vi "Main Editor UI.vi"() -> ()   [LabVIEW 2014, in "Shared Memory editor node.lvclass"]
doc: "This is the main view for configuration the behavior of a module in the DCAF standard editor."
uses:
  Shared Memory editor node.lvclass
  <vilib>/NI/Configuration Framework/Node/NodeRef.ctl
  <vilib>/NI/Configuration Framework/Node/NISE_CEF_Node.lvclass
  <vilib>/NI/AMC/Message Queue.ctl
  <vilib>/NI/AMC/Message.ctl
  <vilib>/NI/Tools/Keyed Array/KeyedArray.ctl
  <vilib>/NI/Configuration Framework/Node/UserEventRef.ctl
  <vilib>/NI/Configuration Framework/Controls/EventCluster.ctl
  <vilib>/NI/DCAF UI Toolkit/Controls/Configure.ctl
  <vilib>/NI/DCAF UI Toolkit/Controls/Add.ctl
  <vilib>/NI/DCAF UI Toolkit/Controls/Remove.ctl
  <vilib>/NI/Configuration Framework/Node/StopEvent.ctl
  <vilib>/NI/Configuration Framework/Node/RefreshUIEvent.ctl
  <vilib>/NI/Configuration Framework/Node/CacheState.ctl
  <vilib>/NI/Configuration Framework/Node/NodeChangeEvent.ctl
  <vilib>/NI/Tag Bus/tag/Data Type.ctl
  Permissions Enum.ctl
  <vilib>/NI/DCAF/Tag Editor Core/Table API/Available Tag Menu/channel action event.ctl
  <vilib>/NI/DCAF/Tag Editor Core/Table API/Available Tag Menu/dialog output action.ctl
  <vilib>/NI/Tag Bus Module Framework/channel/TBM channel.lvclass
  <vilib>/NI/Tag Bus/tag/tag descriptor.lvclass
  <vilib>/NI/DCAF/Tag Editor Core/Table API/Table Manager/Call Back Ref Type Def.ctl
  <vilib>/NI/DCAF/Tag Editor Core/Configuration Editor/Classes/Engine Parent/Engine Parent Editor Node.lvclass
  <vilib>/NI/DCAF/Tag Editor Core/Configuration Editor/Classes/Module editor node/module editor node.lvclass
  sync/sync item.ctl
  sync/sync mechanism.ctl
  <vilib>/NI/DCAF UI Toolkit/Controls/Move One Left.ctl
  <vilib>/NI/DCAF UI Toolkit/Controls/Move One Right.ctl
  <vilib>/NI/DCAF/Tag Editor Core/Table API/Table Manager/references.ctl
  ui controls sync.ctl
  ui controls config.ctl
  ui controls header.ctl
  <vilib>/NI/Tag Bus Module Framework/channel/channel classification.ctl
  <vilib>/Utility/miscctls.llb/LVPositionTypeDef.ctl
  <vilib>/NI/DCAF/Tag Editor Core/Configuration Editor/Classes/Engine Parent/read engine configuration.vi
  <vilib>/NI/Module Execution Interface/Engine Configuration/engine configuration.lvclass
  <vilib>/NI/DCAF/Tag Editor Core/Table API/Listbox/Multi Column Listbox.lvclass
  <vilib>/NI/Configuration Framework/NISE_CEF_TreeControl.lvlib
  <vilib>/NI/Tools/Keyed Array/Tools_KeyedArray.lvlib
  <vilib>/NI/AMC/AMC.lvlib
  <vilib>/NI/DCAF/Tag Editor Core/Table API/Table Manager.lvlib
  <vilib>/NI/DCAF/Tag Editor Core/Table API/Table Manager/Table Manager.lvclass
  <vilib>/NI/DCAF UI Toolkit/Controls/DCAF UI Elements.lvlib
  module/configuration/Shared Memory configuration.lvclass
panel:
  in  "user event out":refnum<user-event>
  in  "Permissions":T1=enum."Read from Memory"
  in  "data type":T2
  in  "node change":T3
  in  "cache state":T4
  in  "refresh UI":T5
  in  "stop event":T6
  in  "Tab Control":T7(tab)
  in  "to shm list":i32(listbox)
  in  "from shm list":i32(listbox)
  in  "add to":T8
  in  "remove to":T9
  in  "add from":T8
  in  "remove from":T9
  in  "avail tags":i32(listbox)
  in  "View":enum32{"From Shared Memory", "To Shared Memory"}(radio)
  in  "Timeout (us)":u32 step=25
  in  "sync end of cycle":T10[](array[typedef])
  in  "Include start time":bool
  out "Shared memory name":string
  out "Struct prototype":string
  in  "sync start of cycle":T10[](array[typedef])
  out "Struct name":string
  in  "Enable sync":bool
  out "C Header File Preview":string
  out "build":u16
  out "fix":u16
  out "minor":u16
  out "major":u16=1
  in  "Generate Header":bool
  in  "output file path":path caption="Output File Path"
  in  "output file string":string caption="output file string (optional)"
  in  "input file string":string caption="input file string (optional)"
  in  "Remove Button":T12
  in  "Add Button":T13
  in  "Table":i32(listbox)
  in  "settings":T14
  in  "user event":T15
  in  "main queue":T16
  in  "node ref":T17
  # "Start of cycle"
  # "End of cycle (optional response)"
  # "Mechanism"
  # "Name in struct"
  # "Mechanism"
  # "Name in struct"
  # "C Header File Generation"
  # "Version"
  # "Shared Memory Files (<EngineName>_<\"input/output\">_<DataType>_<FileString>)"
  # "The data file names will follow a fixed format with an optional appended user file name string. File input and output classification is from the perspective of an  external process (or application) which will access the file.\n\nExample: A C application running in parallel to the DCAF based LabVIEW Real-Time EXE application will view any file that it writes to as an \"output\" data file in Linux shared memory."
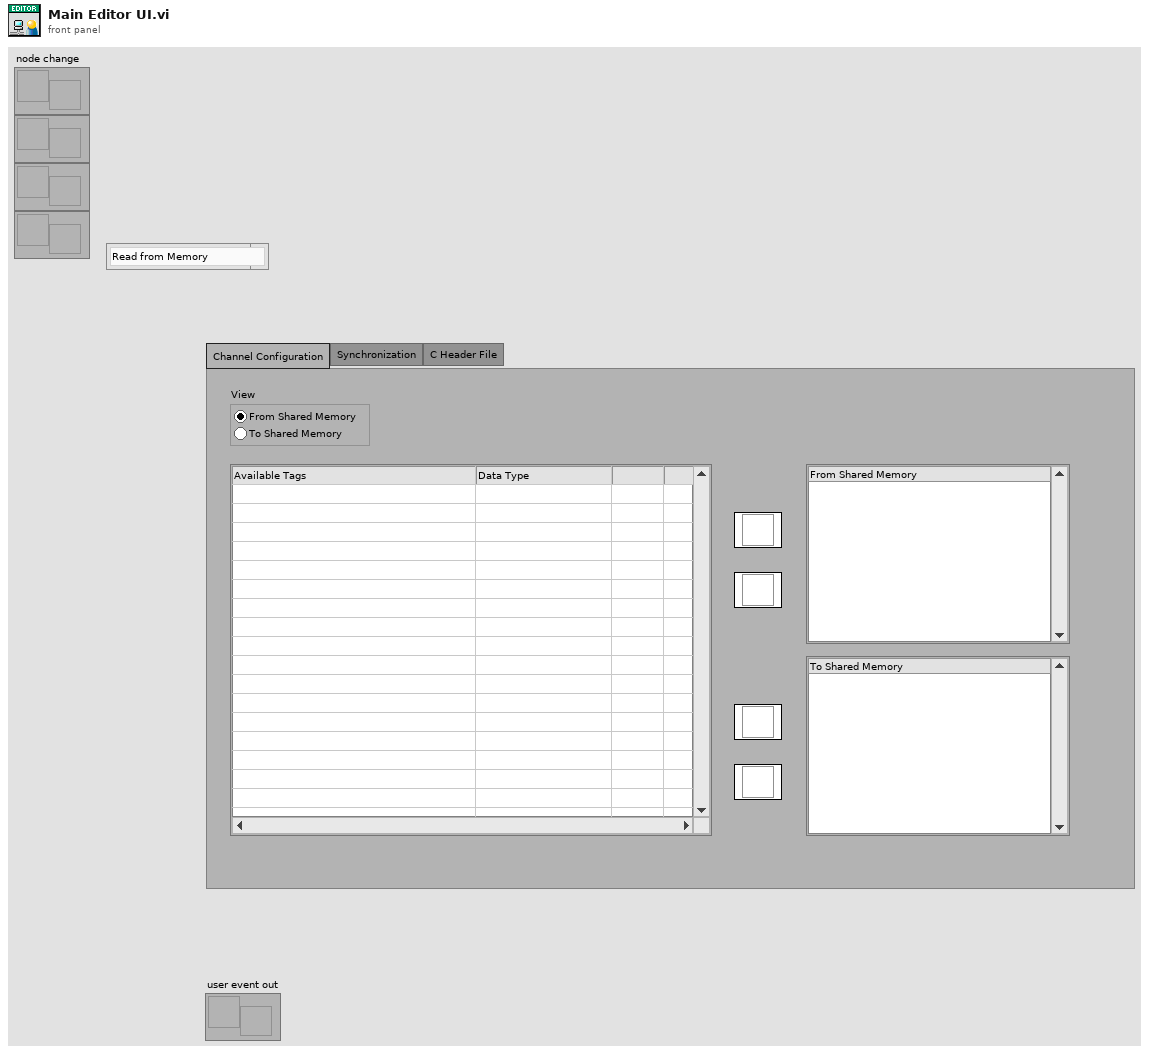
[diagram p1: front panel]
types:
  T1 = typedef "Shared Memory editor node.lvclass/Permissions Enum.ctl" = enum16{"Write to Memory", "Read from Memory"}
  T2 = typedef "tag bus.lvlib/tag descriptor.lvclass/Data Type.ctl" = enum16{"Double", "Single", "I64", "I32", "I16", "I8", "U64", "U32", "U16", "U8", "Boolean", "String", "Array of Double", "Array of Single", "Array of I64", "Array of I32", "Array of I16", "Array of I8", "Array of U64", "Array of U32", "Array of U16", "Array of U8", "Array of Boolean", "Array of String"}
  T3 = typedef "NISE_CEF_Node.lvclass/NodeChangeEvent.ctl" = refnum<user-event>
  T4 = typedef "NISE_CEF_Node.lvclass/CacheState.ctl" = refnum<user-event>
  T5 = typedef "NISE_CEF_Node.lvclass/RefreshUIEvent.ctl" = refnum<user-event>
  T6 = typedef "NISE_CEF_Node.lvclass/StopEvent.ctl" = refnum<user-event>
  T7 = enum32{"Channel Configuration", "Synchronization", "C Header File", "Memory Configuration", "Channel Configuration (old)"}
  T8 = typedef "DCAF UI Elements.lvlib/Move One Right.ctl" = bool
  T9 = typedef "DCAF UI Elements.lvlib/Move One Left.ctl" = bool
  T10 = typedef "Shared Memory configuration.lvclass/sync item.ctl" = cluster{"mechanism":T11, "name":string}
  T11 = typedef "Shared Memory configuration.lvclass/sync mechanism.ctl" = enum16{"Semaphore"}
  T12 = typedef "DCAF UI Elements.lvlib/Remove.ctl" = bool
  T13 = typedef "DCAF UI Elements.lvlib/Add.ctl" = bool
  T14 = typedef "DCAF UI Elements.lvlib/Configure.ctl" = bool
  T15 = typedef "NISE_CEF_Node.lvclass/UserEventRef.ctl" = refnum<user-event>
  T16 = typedef "AMC.lvlib/Message Queue.ctl" = refnum<queue>
  T17 = typedef "NISE_CEF_Node.lvclass/NodeRef.ctl" = refnum<data-value>
  T18 = typedef "Shared Memory editor node.lvclass/ui controls header.ctl" = cluster{"major":refnum<vi>, "minor":refnum<vi>, "fix":refnum<vi>, "build":refnum<vi>, "file path":refnum<vi>, "file preview":refnum<vi>}
  T19 = typedef "Shared Memory editor node.lvclass/ui controls config.ctl" = cluster{"avail tags":refnum<vi>, "from shm list":refnum<vi>, "to shm list":refnum<vi>, "view":refnum<vi>, "add to":refnum<vi>, "add from":refnum<vi>, "remove to":refnum<vi>, "remove from":refnum<vi>}
  T20 = typedef "Shared Memory editor node.lvclass/ui controls sync.ctl" = cluster{"struct name":refnum<vi>, "timeout":refnum<vi>, "shm name":refnum<vi>, "sync end of cycle":refnum<vi>, "sync start of cycle":refnum<vi>, "enable sync":refnum<vi>, "include start time":refnum<vi>, "struct prototype":refnum<vi>}
  T21 = typedef "Table Manager.lvlib/Table Manager.lvclass/references.ctl" = cluster{"stop event":T6, "refresh UI":T5, "cache state":T4, "node change":T3, "user event out":refnum<user-event>, "main queue":T16, "user event":T15}
  T22 = typedef "LVPositionTypeDef.ctl" = cluster{"Left":i32, "Top":i32}
  T23 = typedef "Table Manager.lvlib/Table Manager.lvclass/object ref.ctl" = cluster{"engine":refnum<data-value>, "Node Ref":refnum<data-value>}
  T24 = typedef "Table Manager.lvlib/Column.lvclass/Column Descriptor.ctl" = cluster{"name":string, "caption":string, "Column Type":T25, "Params":string, "AutoSizeMode":i32, "FillWeight":sgl, "MinWidth":u32, "tooltip":string, "Enum Reference":refnum<vi>, "Channel suffix":string, "Read Only":bool, "Call Back VI":T26, "DT Dependency":i32, "name dependency":i32, "data type":T2, "Custom Column":refnum<class "Column.lvclass">}
  T25 = typedef "Table Manager.lvlib/Column.lvclass/Column Type.ctl" = enum16{"String", "Mapping", "Enum", "Custom"}
  T26 = typedef "Table Manager.lvlib/Table Manager.lvclass/Call Back Ref Type Def.ctl" = refnum<vi>
  T27 = typedef "Table Manager.lvlib/Table Manager.lvclass/Table Events.ctl" = cluster{"Menu Selection":refnum<user-event>}
  T28 = typedef "TBM channel.lvclass/channel classification.ctl" = enum16{"input data", "output data", "processing parameter", "processing result"}
  T29 = enum8{"Enabled", "Disabled", "Disabled and Grayed Out"}
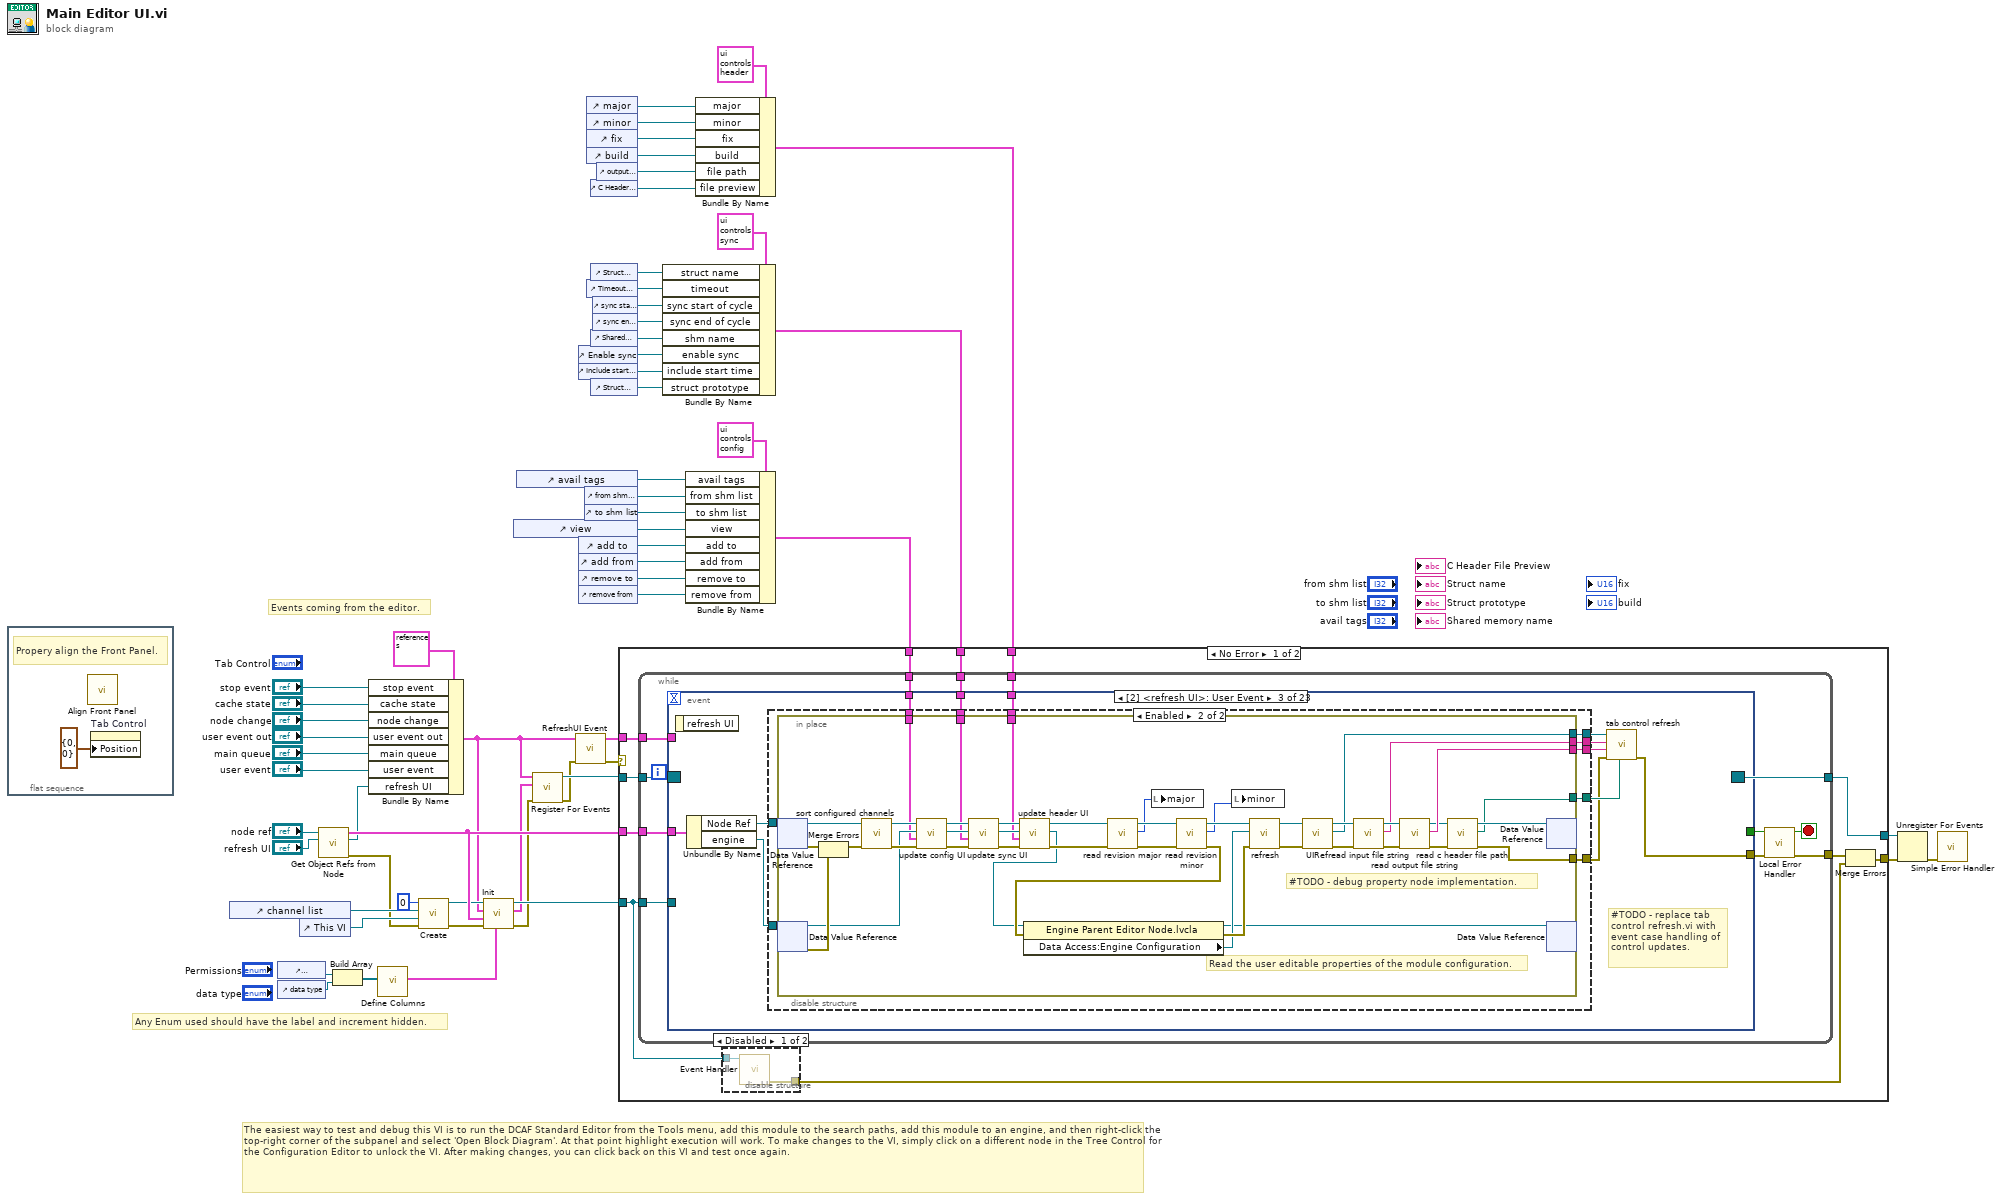
[diagram p0: block diagram]
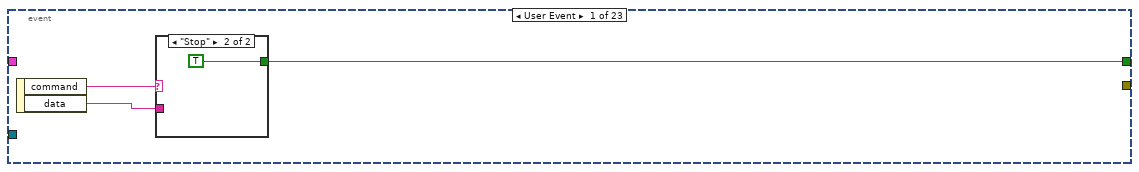
[diagram p3: hidden frame]
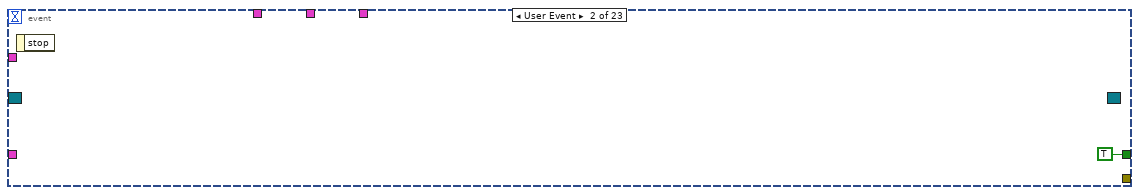
[diagram p5: hidden frame]
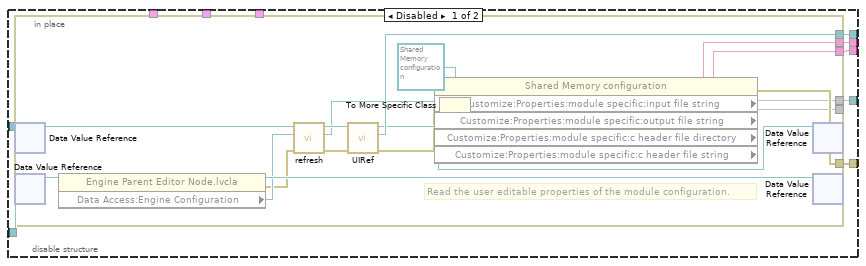
[diagram p6: hidden frame]
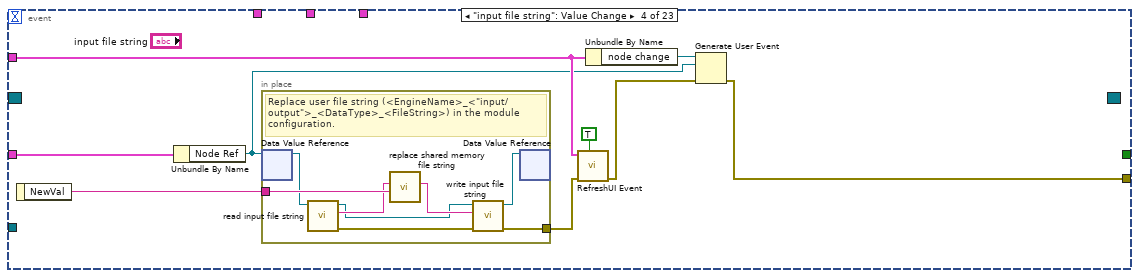
[diagram p7: hidden frame]
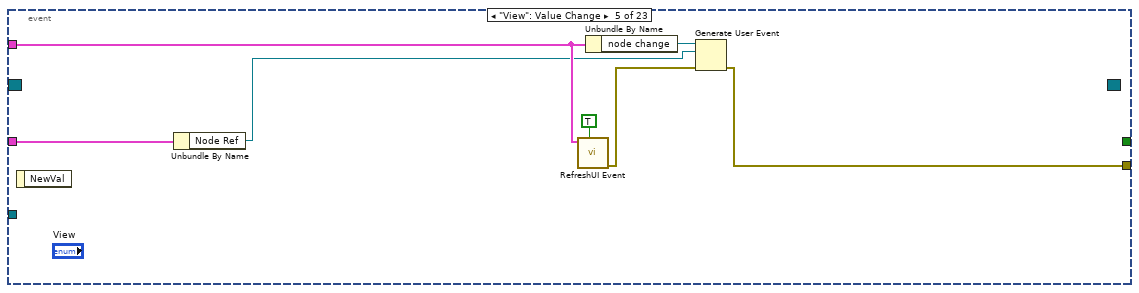
[diagram p8: hidden frame]
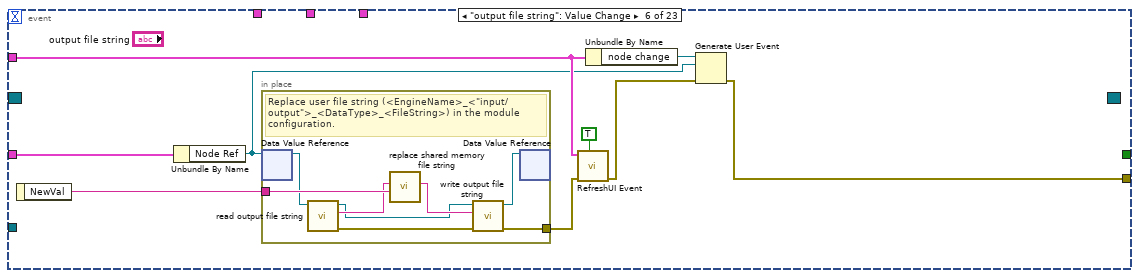
[diagram p9: hidden frame]
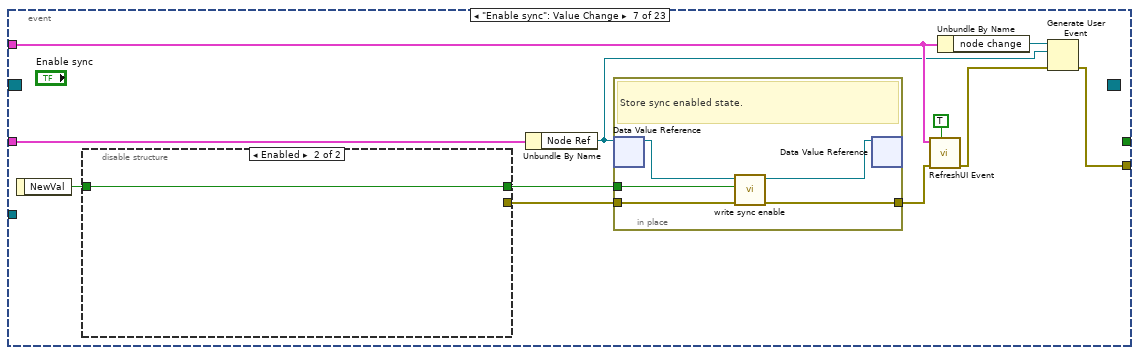
[diagram p10: hidden frame]
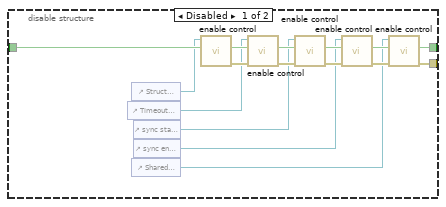
[diagram p11: hidden frame]
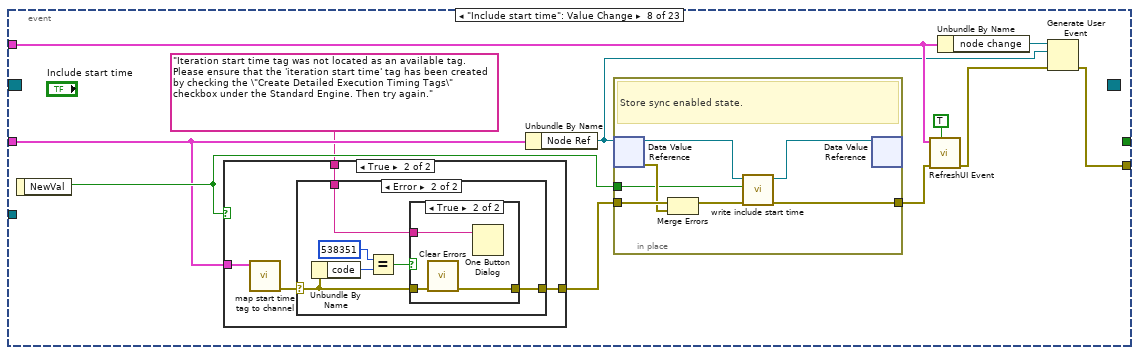
[diagram p12: hidden frame]
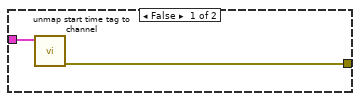
[diagram p13: hidden frame]
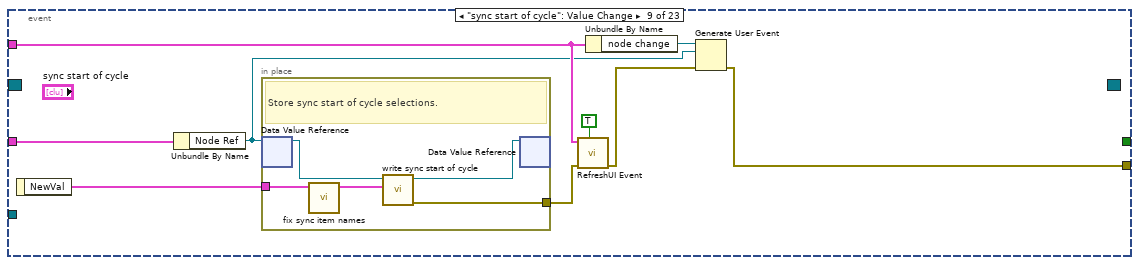
[diagram p16: hidden frame]
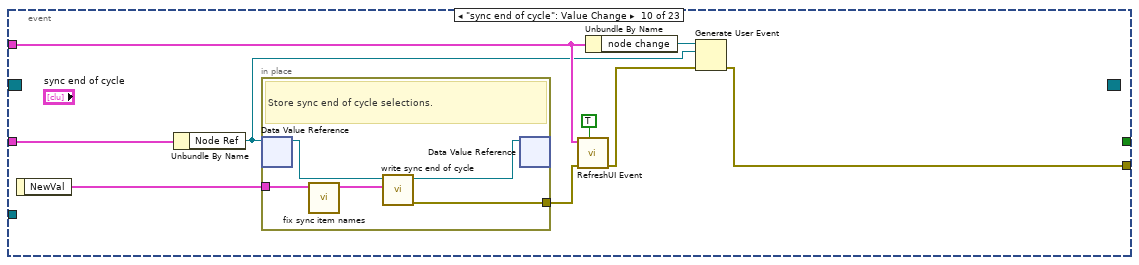
[diagram p17: hidden frame]
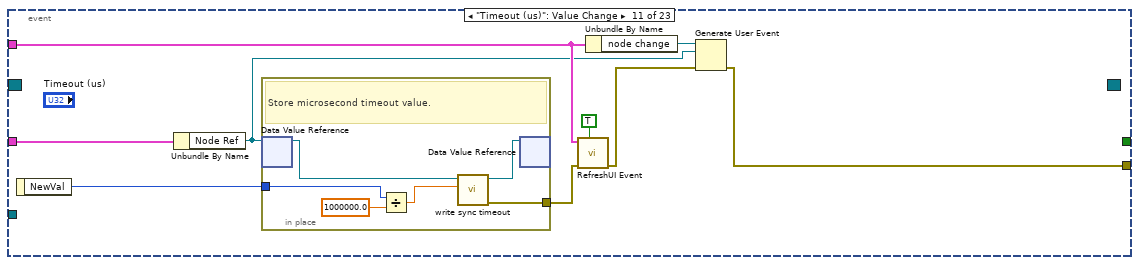
[diagram p18: hidden frame]
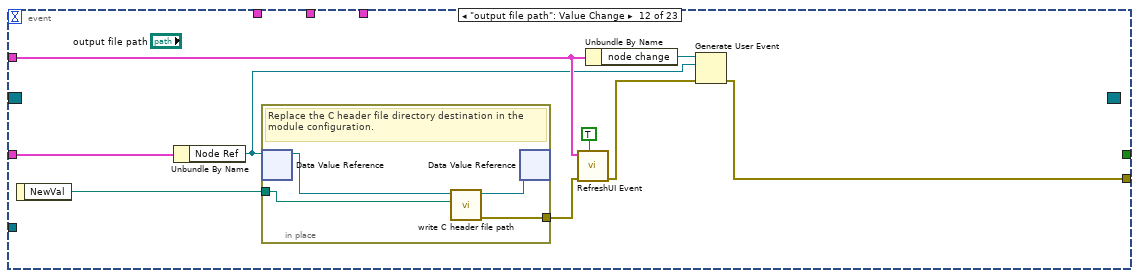
[diagram p19: hidden frame]
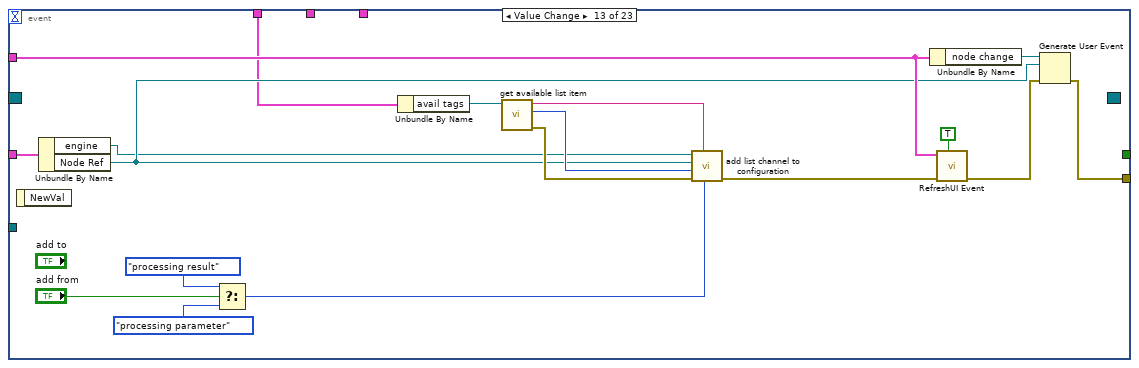
[diagram p20: hidden frame]
diagram:
  # "The easiest way to test and debug this VI is to run the DCAF Standard Editor from the Tools menu, add this module to the search paths, add this module to an engine, and then right-click the top-right corner of the subpanel and select 'Open Block Diagram'. At that point highlight execution will work. To make changes to the VI, simply click on a different node in the Tree Control for the Configuration Editor to unlock the VI. After making changes, you can click back on this VI and test once again."
  # "Any Enum used should have the label and increment hidden."
  # "Events coming from the editor."
  n1 = flat-sequence {
    frame #0 {
      # "Propery align the Front Panel."
      n2 = call <vilib>:"Align Front Panel.vi"() -> ()  [unwired: 10 in, 2 out]
      n3 = property on="Tab Control" class="TabCtl (strict)"("Position"=T22 {"Left"=0, "Top"=0}) -> ()  [unwired: 2 in, 2 out]
    }
  }
  n4 = control-ref of="channel list"() -> (w37:refnum<vi>)
  n5 = control-ref of="Permissions"() -> (w47:refnum<vi>)
  n6 = control-ref of="data type"() -> (w46:refnum<vi>)
  n7 = control-ref of="This VI"() -> (w35:refnum<vi>)
  n8 = call "Get Object Refs from Node.vi"("Refresh UI"="refresh UI", "Data Value Reference in"="node ref") -> ("error out"=w32:errorcluster, "Refresh UI out"=w30:T5, "References"=w44:T23)  [unwired: 7 in]
  n9 = Build Array(w47, w46) -> (w45:refnum<vi>[])
  n10 = Bundle By Name(cluster=T21 {"stop event"=refnum, "refresh UI"=refnum, "cache state"=refnum, "node change"=refnum, "user event out"=refnum, "main queue"=refnum, "user event"=refnum} ("References"), "stop event"="stop event", "cache state"="cache state", "node change"="node change", "user event out"="user event out", "main queue"="main queue", "user event"="user event", "refresh UI"=w30) -> (w29:T21)
  n11 = call "Define Columns.vi"("Enum Array"=w45) -> ("Column Definition"=w49:T24[])  [unwired: 10 in]
  n12 = call <vilib>:"Create.vi"("error in (no error)"=w32, "Top VI"=w35, "Listbox"=w37, "Index"=0) -> ("error out"=w33:errorcluster, "reference out"=w34:refnum<class "Multi Column Listbox.lvclass">)  [unwired: 6 in]
  n13 = call-dynamic "Init.vi"("Column Descriptors"=w49, "error in (no error)"=w33, "Node object refs"=w44, "Event References"=w29, "Multi Column Listbox in"=w34) -> ("error out"=w39:errorcluster, "Table Events"=w38:T27, "Multi Column Listbox out"=w43:refnum<class "Multi Column Listbox.lvclass">)  [unwired: 4 in]
  n14 = control-ref of="view"() -> (w13:refnum<vi>)
  n15 = control-ref of="avail tags"() -> (w17:refnum<vi>)
  n16 = call "Register For Events.vi"("error in"=w39, "Table Events"=w38, "References"=w29) -> ("error out"=w41:errorcluster, "Event Registration Refnum"=w50:refnum<event-registration>)  [unwired: 7 in]
  n17 = call "RefreshUI Event.vi"("error in (no error)"=w41, "References in"=w29) -> ("error out"=w40:errorcluster, "References out"=w48:T21)  [unwired: 8 in]
  n18 = control-ref of="Enable sync"() -> (w26:refnum<vi>)
  n19 = control-ref of="Include start time"() -> (w21:refnum<vi>)
  n20 = control-ref of="add to"() -> (w12:refnum<vi>)
  n21 = control-ref of="add from"() -> (w11:refnum<vi>)
  n22 = control-ref of="remove to"() -> (w10:refnum<vi>)
  n23 = control-ref of="remove from"() -> (w9:refnum<vi>)
  n24 = control-ref of="from shm list"() -> (w16:refnum<vi>)
  n25 = control-ref of="to shm list"() -> (w15:refnum<vi>)
  n26 = control-ref of="major"() -> (w5:refnum<vi>)
  n27 = control-ref of="minor"() -> (w6:refnum<vi>)
  n28 = control-ref of="fix"() -> (w3:refnum<vi>)
  n29 = control-ref of="build"() -> (w4:refnum<vi>)
  n30 = control-ref of="Timeout (us)"() -> (w19:refnum<vi>)
  n31 = control-ref of="C Header File Preview"() -> (w1:refnum<vi>)
  n32 = control-ref of="Struct name"() -> (w27:refnum<vi>)
  n33 = control-ref of="Shared memory name"() -> (w25:refnum<vi>)
  n34 = control-ref of="Struct prototype"() -> (w20:refnum<vi>)
  n35 = control-ref of="sync start of cycle"() -> (w23:refnum<vi>)
  n36 = control-ref of="sync end of cycle"() -> (w24:refnum<vi>)
  n37 = control-ref of="output file path"() -> (w7:refnum<vi>)
  n38 = Bundle By Name(cluster=T20 {"struct name"=refnum, "timeout"=refnum, "shm name"=refnum, "sync end of cycle"=refnum, "sync start of cycle"=refnum, "enable sync"=refnum, "include start time"=refnum, "struct prototype"=refnum} ("sync ui refs"), "struct name"=w27, "timeout"=w19, "sync start of cycle"=w23, "sync end of cycle"=w24, "shm name"=w25, "enable sync"=w26, "include start time"=w21, "struct prototype"=w20) -> (w22:T20)
  n39 = Bundle By Name(cluster=T19 {"avail tags"=refnum, "from shm list"=refnum, "to shm list"=refnum, "view"=refnum, "add to"=refnum, "add from"=refnum, "remove to"=refnum, "remove from"=refnum} ("config ui refs"), "avail tags"=w17, "from shm list"=w16, "to shm list"=w15, "view"=w13, "add to"=w12, "add from"=w11, "remove to"=w10, "remove from"=w9) -> (w14:T19)
  n40 = Bundle By Name(cluster=T18 {"major"=refnum, "minor"=refnum, "fix"=refnum, "build"=refnum, "file path"=refnum, "file preview"=refnum} ("header ui refs"), "major"=w5, "minor"=w6, "fix"=w3, "build"=w4, "file path"=w7, "file preview"=w1) -> (w2:T18)
  n41 = case shown="No Error" w40 {
    selector: w40 -> [_ w508]
    tunnel: w50 -> [w72 w507]
    tunnel: [w71 w507] -> w60
    tunnel: [w65 w508] -> w59
    tunnel: w48 -> [w70 _]
    tunnel: w44 -> [w69 _]
    tunnel: w43 -> [w68 _]
    tunnel: w22 -> [w64 _]
    tunnel: w14 -> [w63 _]
    tunnel: w2 -> [w62 _]
    frame No Error {
      n42 = while {
        tunnel: w72 -> [w86]
        tunnel: [w85] -> w71
        tunnel: [w82] -> w66
        tunnel: w70 -> [w80]
        tunnel: w69 -> [w79]
        tunnel: w68 -> [w78]
        tunnel: w64 -> [w77]
        tunnel: w63 -> [w76]
        tunnel: w62 -> [w75]
        stop <- w84 stop-if-true
        n43 = event shown="[2] <refresh UI>: User Event" {
          selector: w86 -> [_ _ _ _ _ _ _ _ _ _ _ _ _ _ _ _ _ _ _ _ _ _ _]
          dyn-events: [_ _ _ _ _ _ _ _ _ _ _ _ _ _ _ _ _ _ _ _ _ _ _] -> w85
          timeout: _ -> [_ _ _ _ _ _ _ _ _ _ _ _ _ _ _ _ _ _ _ _ _ _ _]
          tunnel: [w89 TRUE _ _ _ _ _ _ _ _ _ _ _ _ _ _ _ FALSE _ _ _ _ _] -> w83
          tunnel: [_ _ w95 w182 w199 w206 w227 w261 w291 w305 w319 w335 w358 w376 w391 w405 w418 _ w457 w464 w481 w489 _] -> w81
          tunnel: w80 -> [_ _ _ w186 w203 w210 w231 w265 w295 w309 w323 w337 w360 w378 w392 w406 w420 w453 w461 w475 w483 w485 _]
          tunnel: w79 -> [_ _ w96 w188 w204 w212 w232 w258 w297 w311 w325 w340 w362 w380 w395 w409 w425 _ w462 w474 w479 w486 _]
          tunnel: w78 -> [_ _ _ _ _ _ _ _ _ _ _ _ _ _ _ _ _ _ _ w470 w480 _ _]
          tunnel: w77 -> [_ _ w94 _ _ _ _ _ _ _ _ _ _ _ _ _ _ _ _ _ _ _ _]
          tunnel: w76 -> [_ _ w93 _ _ _ _ _ _ _ _ _ w347 w375 _ _ _ _ _ _ _ _ _]
          tunnel: w75 -> [_ _ w92 _ _ _ _ _ _ _ _ _ _ _ _ _ _ _ _ _ _ _ _]
          event User Event {
            n44 = event-data() -> ("command"=w88:string, "data"=w87:string)  [unwired: 1 in]
            n45 = case shown="\"Stop\"" w88 {
              tunnel: [_ TRUE] -> w89
              tunnel: w87 -> [_ _]
              frame Default {
              }
              frame "Stop" {
              }
            }
          }
          event User Event {
            n46 = event-data() -> ()  [unwired: 1 in, 1 out]
          }
          event User Event {
            # "#TODO - replace tab\ncontrol refresh.vi with\nevent case handling of\ncontrol updates."
            n47 = event-data() -> ()  [unwired: 1 in, 1 out]
            n48 = Unbundle By Name(w96) -> ("Node Ref"=w97:refnum<data-value>, "engine"=w98:refnum<data-value>)
            n49 = disable-structure shown="Enabled" {
              disable-tunnel: [w110 w139] -> w103
              disable-tunnel: [w109 w133] -> w102
              disable-tunnel: [w108 w134] -> w101
              disable-tunnel: [w107 w135] -> w100
              disable-tunnel: [w106 w136] -> w99
              disable-tunnel: w98 -> [w105 w138]
              disable-tunnel: w97 -> [w104 w137]
              disable-tunnel: w94 -> [_ w132]
              disable-tunnel: w93 -> [_ w131]
              disable-tunnel: w92 -> [_ w130]
              frame Disabled {
                n50 = in-place {
                  in-place-border: [w128] -> w106
                  in-place-border: [w127] -> w110
                  in-place-border: [w126] -> w107
                  in-place-border: [w125] -> w108
                  in-place-border: [w124] -> w109
                  in-place-border: [w123] -> _
                  # "Read the user editable properties of the module configuration."
                  n51 = in-place-dvr #1(w104) -> (w120:refnum<class "module editor node.lvclass">)  [unwired: 1 out]
                  n52 = in-place-dvr #2(w105) -> (w129:refnum<class "Engine Parent Editor Node.lvclass">)  [unwired: 1 out]
                  n53 = property class="Engine Parent Editor Node.lvcla"(reference=w129) -> (reference out=w121:refnum<class "Engine Parent Editor Node.lvclass">, error out=w117:errorcluster, "Data Access:Engine Configuration"=w118:refnum<class "engine configuration.lvclass">)  [unwired: 1 in]
                  n54 = call-dynamic "refresh.vi"("error in (no error)"=w117, "Engine Configuration In"=w118, "Module Editor Node In"=w120) -> ("error out"=w116:errorcluster, "Engine Configuration Out"=w112:refnum<class "engine configuration.lvclass">, "Module Editor Node Out"=w119:refnum<class "module editor node.lvclass">)  [unwired: 6 in]
                  n55 = call-dynamic "UIRef.vi"("error in"=w116, "node in"=w119) -> ("error out"=w111:errorcluster, "VI refnum"=w127:refnum<vi>, "node out"=w122:refnum<class "module editor node.lvclass">)  [unwired: 7 in]
                  n56 = To More Specific Class(target class=refnum<class "Shared Memory configuration.lvclass"> refnum ("shared memory configuration"), reference=w112, error in=w111) -> (specific class reference=w114:refnum<class "Shared Memory configuration.lvclass">, error out=w113:errorcluster)
                  n57 = property class="Shared Memory configuration"(reference=w114, error in=w113) -> (error out=w128:errorcluster, "Customize:Properties:module specific:input file string"=w126:string, "Customize:Properties:module specific:output file string"=w125:string, "Customize:Properties:module specific:c header file directory"=w124, "Customize:Properties:module specific:c header file string"=w123)  [unwired: 1 out]
                  n58 = in-place-dvr #1(w122) -> ()  [unwired: 2 out]
                  n59 = in-place-dvr #2(w121) -> ()  [unwired: 2 out]
                }
              }
              frame Enabled {
                n60 = in-place {
                  in-place-border: [w172] -> w139
                  in-place-border: [w160] -> w136
                  in-place-border: [w174] -> w135
                  in-place-border: [w173] -> w134
                  in-place-border: [w157] -> w133
                  in-place-border: w132 -> [w144]
                  in-place-border: w131 -> [w143]
                  in-place-border: w130 -> [w145]
                  # "#TODO - debug property node implementation."
                  # "Read the user editable properties of the module configuration."
                  n61 = in-place-dvr #3(w137) -> (w155:refnum<class "module editor node.lvclass">, w169:errorcluster)
                  n62 = in-place-dvr #4(w138) -> (w149:refnum<class "Engine Parent Editor Node.lvclass">, w168:errorcluster)
                  n63 = Merge Errors(w169, w168) -> (w154:errorcluster)
                  n64 = call "sort configured channels.vi"("error in"=w154, "shared memory editor node"=w155) -> ("error out"=w153:errorcluster, "shared memory editor node out"=w152:refnum<class "module editor node.lvclass">)  [unwired: 8 in]
                  n65 = call "update config UI.vi"("error in (no error)"=w153, "config ui refs"=w143, "engine in"=w149, "shared memory editor node in"=w152) -> ("error out"=w156:errorcluster, "engine out"=w150:refnum<class "Engine Parent Editor Node.lvclass">, "shared memory editor node out"=w151:refnum<class "module editor node.lvclass">)  [unwired: 5 in]
                  n66 = call "update sync UI.vi"("error in (no error)"=w156, "sync ui refs"=w144, "engine in"=w150, "shared memory editor node in"=w151) -> ("error out"=w147:errorcluster, "engine out"=w146:refnum<class "Engine Parent Editor Node.lvclass">, "shared memory editor node out"=w148:refnum<class "module editor node.lvclass">)  [unwired: 5 in]
                  n67 = call "update header UI.vi"("error in (no error)"=w147, "header ui refs"=w145, "engine in"=w146, "shared memory editor node in"=w148) -> ("error out"=w142:errorcluster, "engine out"=w140:refnum<class "Engine Parent Editor Node.lvclass">, "shared memory editor node out"=w141:refnum<class "module editor node.lvclass">)  [unwired: 5 in]
                  n68 = call "read revision major.vi"("error in"=w142, "shared memory editor node"=w141) -> ("error out"=w167:errorcluster, "revision major"=w163:u16, "shared memory editor node out"=w164:refnum<class "module editor node.lvclass">)  [unwired: 7 in]
                  n69 = local write "major"(w163) -> ()
                  n70 = call "read revision minor.vi"("error in"=w167, "shared memory editor node"=w164) -> ("error out"=w165:errorcluster, "revision minor"=w162:u16, "shared memory editor node out"=w166:refnum<class "module editor node.lvclass">)  [unwired: 7 in]
                  n71 = property class="Engine Parent Editor Node.lvcla"(reference=w140, error in=w165) -> (reference out=w170:refnum<class "Engine Parent Editor Node.lvclass">, error out=w180:errorcluster, "Data Access:Engine Configuration"=w171:refnum<class "engine configuration.lvclass">)
                  n72 = local write "minor"(w162) -> ()
                  n73 = call-dynamic "refresh.vi"("error in (no error)"=w180, "Engine Configuration In"=w171, "Module Editor Node In"=w166) -> ("error out"=w179:errorcluster, "Module Editor Node Out"=w181:refnum<class "module editor node.lvclass">)  [unwired: 6 in, 1 out]
                  n74 = call-dynamic "UIRef.vi"("error in"=w179, "node in"=w181) -> ("error out"=w176:errorcluster, "VI refnum"=w172:refnum<vi>, "node out"=w177:refnum<class "module editor node.lvclass">)  [unwired: 7 in]
                  n75 = call "read input file string.vi"("error in"=w176, "shared memory editor node"=w177) -> ("error out"=w175:errorcluster, "input file string"=w174:string, "shared memory editor node out"=w178:refnum<class "module editor node.lvclass">)  [unwired: 7 in]
                  n76 = call "read output file string.vi"("error in"=w175, "shared memory editor node"=w178) -> ("error out"=w161:errorcluster, "output file string"=w173:string, "shared memory editor node out"=w158:refnum<class "module editor node.lvclass">)  [unwired: 7 in]
                  n77 = call "read c header file path.vi"("error in"=w161, "shared memory editor node"=w158) -> ("error out"=w160:errorcluster, "c header file path"=w157:path, "shared memory editor node out"=w159:refnum<class "module editor node.lvclass">)  [unwired: 7 in]
                  n78 = in-place-dvr #3(w159) -> ()  [unwired: 2 out]
                  n79 = in-place-dvr #4(w170) -> ()  [unwired: 2 out]
                }
              }
            }
            n80 = call "tab control refresh.vi"("c header file path"=w102, "error in"=w99, "output file string"=w101, "input file string"=w100, "VI reference"=w103) -> ("error out"=w95:errorcluster)  [unwired: 6 in]
          }
          event "input file string": Value Change {
            n81 = event-data() -> ("NewVal"=w187:string)  [unwired: 1 in]
            n82 = Unbundle By Name(w188) -> ("Node Ref"=w184:refnum<data-value>)
            n83 = in-place {
              in-place-border: w187 -> [w195]
              in-place-border: [w196] -> w190
              # "Replace user file string (<EngineName>_<\"input/output\">_<DataType>_<FileString>) in the module configuration."
              n84 = in-place-dvr #5(w184) -> (w193:refnum<class "module editor node.lvclass">)  [unwired: 1 out]
              n85 = call "read input file string.vi"("shared memory editor node"=w193) -> ("error out"=w197:errorcluster, "input file string"=w194:string, "shared memory editor node out"=w191:refnum<class "module editor node.lvclass">)  [unwired: 8 in]
              n86 = call "replace shared memory file string.vi"("new string"=w195, "file name"=w194) -> ("new file name"=w192:string)  [unwired: 9 in]
              n87 = call "write input file string.vi"("error in"=w197, "input file string"=w192, "shared memory editor node"=w191) -> ("error out"=w196:errorcluster, "shared memory editor node out"=w198:refnum<class "module editor node.lvclass">)  [unwired: 7 in]
              n88 = in-place-dvr #5(w198) -> ()  [unwired: 2 out]
            }
            n89 = call "RefreshUI Event.vi"("Refresh (T)"=TRUE, "error in (no error)"=w190, "References in"=w186) -> ("error out"=w183:errorcluster)  [unwired: 7 in, 1 out]
            n90 = Unbundle By Name(w186) -> ("node change"=w185:T3)
            n91 = Generate User Event(user event=w185, event data cluster=w184, error in=w183) -> (error out=w182:errorcluster)  [unwired: 1 in, 1 out]
          }
          event "View": Value Change {
            n92 = event-data() -> ()  [unwired: 1 in, 1 out]
            n93 = Unbundle By Name(w204) -> ("Node Ref"=w201:refnum<data-value>)
            n94 = call "RefreshUI Event.vi"("Refresh (T)"=TRUE, "References in"=w203) -> ("error out"=w200:errorcluster)  [unwired: 8 in, 1 out]
            n95 = Unbundle By Name(w203) -> ("node change"=w202:T3)
            n96 = Generate User Event(user event=w202, event data cluster=w201, error in=w200) -> (error out=w199:errorcluster)  [unwired: 1 in, 1 out]
          }
          event "output file string": Value Change {
            n97 = event-data() -> ("NewVal"=w211:string)  [unwired: 1 in]
            n98 = Unbundle By Name(w212) -> ("Node Ref"=w208:refnum<data-value>)
            n99 = in-place {
              in-place-border: w211 -> [w219]
              in-place-border: [w220] -> w214
              # "Replace user file string (<EngineName>_<\"input/output\">_<DataType>_<FileString>) in the module configuration."
              n100 = in-place-dvr #6(w208) -> (w217:refnum<class "module editor node.lvclass">)  [unwired: 1 out]
              n101 = call "read output file string.vi"("shared memory editor node"=w217) -> ("error out"=w221:errorcluster, "output file string"=w218:string, "shared memory editor node out"=w215:refnum<class "module editor node.lvclass">)  [unwired: 8 in]
              n102 = call "replace shared memory file string.vi"("new string"=w219, "file name"=w218) -> ("new file name"=w216:string)  [unwired: 9 in]
              n103 = call "write output file string.vi"("error in"=w221, "output file string"=w216, "shared memory editor node"=w215) -> ("error out"=w220:errorcluster, "shared memory editor node out"=w222:refnum<class "module editor node.lvclass">)  [unwired: 7 in]
              n104 = in-place-dvr #6(w222) -> ()  [unwired: 2 out]
            }
            n105 = call "RefreshUI Event.vi"("Refresh (T)"=TRUE, "error in (no error)"=w214, "References in"=w210) -> ("error out"=w207:errorcluster)  [unwired: 7 in, 1 out]
            n106 = Unbundle By Name(w210) -> ("node change"=w209:T3)
            n107 = Generate User Event(user event=w209, event data cluster=w208, error in=w207) -> (error out=w206:errorcluster)  [unwired: 1 in, 1 out]
          }
          event "Enable sync": Value Change {
            n108 = event-data() -> ("NewVal"=w225:bool)  [unwired: 1 in]
            n109 = disable-structure shown="Enabled" {
              disable-tunnel: w225 -> [w242 w250]
              disable-tunnel: [w237 w250] -> w224
              disable-tunnel: [w236 _] -> w223
              frame Disabled {
                n110 = control-ref of="Timeout (us)"() -> (w234:refnum<vi>)
                n111 = control-ref of="Struct name"() -> (w240:refnum<vi>)
                n112 = control-ref of="Shared memory name"() -> (w235:refnum<vi>)
                n113 = control-ref of="sync start of cycle"() -> (w245:refnum<vi>)
                n114 = control-ref of="sync end of cycle"() -> (w244:refnum<vi>)
                n115 = call "enable control.vi"("enabled? (T)"=w242, "control in"=w240) -> ("error out"=w243:errorcluster, "enabled out"=w241:bool)  [unwired: 7 in, 1 out]
                n116 = call "enable control.vi"("error in (no error)"=w243, "enabled? (T)"=w241, "control in"=w234) -> ("error out"=w249:errorcluster, "enabled out"=w247:bool)  [unwired: 6 in, 1 out]
                n117 = call "enable control.vi"("error in (no error)"=w249, "enabled? (T)"=w247, "control in"=w245) -> ("error out"=w248:errorcluster, "enabled out"=w246:bool)  [unwired: 6 in, 1 out]
                n118 = call "enable control.vi"("error in (no error)"=w248, "enabled? (T)"=w246, "control in"=w244) -> ("error out"=w239:errorcluster, "enabled out"=w238:bool)  [unwired: 6 in, 1 out]
                n119 = call "enable control.vi"("error in (no error)"=w239, "enabled? (T)"=w238, "control in"=w235) -> ("error out"=w236:errorcluster, "enabled out"=w237:bool)  [unwired: 6 in, 1 out]
              }
              frame Enabled {
              }
            }
            n120 = Unbundle By Name(w232) -> ("Node Ref"=w229:refnum<data-value>)
            n121 = in-place {
              in-place-border: w224 -> [w252]
              in-place-border: [w255] -> w226
              in-place-border: w223 -> [w251]
              # "Store sync enabled state."
              n122 = in-place-dvr #7(w229) -> (w254:refnum<class "module editor node.lvclass">)  [unwired: 1 out]
              n123 = call "write sync enable.vi"("error in"=w251, "sync enable"=w252, "shared memory editor node"=w254) -> ("error out"=w255:errorcluster, "shared memory editor node out"=w253:refnum<class "module editor node.lvclass">)  [unwired: 7 in]
              n124 = in-place-dvr #7(w253) -> ()  [unwired: 2 out]
            }
            n125 = call "RefreshUI Event.vi"("Refresh (T)"=TRUE, "error in (no error)"=w226, "References in"=w231) -> ("error out"=w228:errorcluster)  [unwired: 7 in, 1 out]
            n126 = Unbundle By Name(w231) -> ("node change"=w230:T3)
            n127 = Generate User Event(user event=w230, event data cluster=w229, error in=w228) -> (error out=w227:errorcluster)  [unwired: 1 in, 1 out]
          }
          event "Include start time": Value Change {
            n128 = event-data() -> ("NewVal"=w259:bool)  [unwired: 1 in]
            n129 = case shown="True" w259 {
              tunnel: w258 -> [w267 w272]
              tunnel: [w268 w270] -> w257
              tunnel: "Iteration start time tag was not located as an available tag. Please ensure that the 'iteration start time' tag has been created by checking the \"Create Detailed Execution Timing Tags\" checkbox under the Standard Engine. Then try again." -> [_ w269]
              frame False {
                n130 = call "unmap start time tag to channel.vi"("References in"=w267) -> ("error out"=w268:errorcluster)  [unwired: 9 in, 1 out]
              }
              frame True {
                n131 = call "map start time tag to channel.vi"("References in"=w272) -> ("error out"=w271:errorcluster)  [unwired: 9 in, 1 out]
                n132 = case shown="Error" w271 {
                  selector: w271 -> [w273 w276]
                  tunnel: [w273 w275] -> w270
                  tunnel: w269 -> [_ w274]
                  frame No Error {
                    # "butterflies and rainbows"
                  }
                  frame Error {
                    n133 = Unbundle By Name(w276) -> ("code"=w279:i32)
                    n134 = Equal?(x=538351, y=w279) -> (x = y?=w277:bool)
                    n135 = case shown="True" w277 {
                      tunnel: w276 -> [w280 w283]
                      tunnel: [w280 w282] -> w275
                      tunnel: w274 -> [_ w281]
                      frame False {
                      }
                      frame True {
                        n136 = call <vilib>:"Clear Errors.vi"("error in (no error)"=w283) -> ("error out"=w282:errorcluster)  [unwired: 5 in, 1 out]
                        n137 = One Button Dialog(message=w281) -> ()  [unwired: 1 in, 1 out]
                      }
                    }
                  }
                }
              }
            }
            n138 = Unbundle By Name(w258) -> ("Node Ref"=w263:refnum<data-value>)
            n139 = in-place {
              in-place-border: [w289] -> w260
              in-place-border: w259 -> [w284]
              in-place-border: w257 -> [w287]
              # "Store sync enabled state."
              n140 = in-place-dvr #8(w263) -> (w288:refnum<class "module editor node.lvclass">, w286:errorcluster)
              n141 = Merge Errors(w287, w286) -> (w285:errorcluster)
              n142 = call "write include start time.vi"("error in"=w285, "include start time"=w284, "shared memory editor node"=w288) -> ("error out"=w289:errorcluster, "shared memory editor node out"=w290:refnum<class "module editor node.lvclass">)  [unwired: 7 in]
              n143 = in-place-dvr #8(w290) -> ()  [unwired: 2 out]
            }
            n144 = call "RefreshUI Event.vi"("Refresh (T)"=TRUE, "error in (no error)"=w260, "References in"=w265) -> ("error out"=w262:errorcluster)  [unwired: 7 in, 1 out]
            n145 = Unbundle By Name(w265) -> ("node change"=w264:T3)
            n146 = Generate User Event(user event=w264, event data cluster=w263, error in=w262) -> (error out=w261:errorcluster)  [unwired: 1 in, 1 out]
          }
          event "sync start of cycle": Value Change {
            n147 = event-data() -> ("NewVal"=w296:T10[])  [unwired: 1 in]
            n148 = Unbundle By Name(w297) -> ("Node Ref"=w293:refnum<data-value>)
            n149 = in-place {
              in-place-border: w296 -> [w301]
              in-place-border: [w304] -> w299
              # "Store sync start of cycle selections."
              n150 = in-place-dvr #9(w293) -> (w302:refnum<class "module editor node.lvclass">)  [unwired: 1 out]
              n151 = call "fix sync item names.vi"("sync items in"=w301) -> ("sync items out"=w300:T10[])  [unwired: 10 in]
              n152 = call "write sync start of cycle.vi"("sync start of cycle"=w300, "shared memory editor node"=w302) -> ("error out"=w304:errorcluster, "shared memory editor node out"=w303:refnum<class "module editor node.lvclass">)  [unwired: 8 in]
              n153 = in-place-dvr #9(w303) -> ()  [unwired: 2 out]
            }
            n154 = call "RefreshUI Event.vi"("Refresh (T)"=TRUE, "error in (no error)"=w299, "References in"=w295) -> ("error out"=w292:errorcluster)  [unwired: 7 in, 1 out]
            n155 = Unbundle By Name(w295) -> ("node change"=w294:T3)
            n156 = Generate User Event(user event=w294, event data cluster=w293, error in=w292) -> (error out=w291:errorcluster)  [unwired: 1 in, 1 out]
          }
          event "sync end of cycle": Value Change {
            n157 = event-data() -> ("NewVal"=w310:T10[])  [unwired: 1 in]
            n158 = Unbundle By Name(w311) -> ("Node Ref"=w307:refnum<data-value>)
            n159 = in-place {
              in-place-border: w310 -> [w315]
              in-place-border: [w318] -> w313
              # "Store sync end of cycle selections."
              n160 = in-place-dvr #10(w307) -> (w316:refnum<class "module editor node.lvclass">)  [unwired: 1 out]
              n161 = call "fix sync item names.vi"("sync items in"=w315) -> ("sync items out"=w314:T10[])  [unwired: 10 in]
              n162 = call "write sync end of cycle.vi"("sync end of cycle"=w314, "shared memory editor node"=w316) -> ("error out"=w318:errorcluster, "shared memory editor node out"=w317:refnum<class "module editor node.lvclass">)  [unwired: 8 in]
              n163 = in-place-dvr #10(w317) -> ()  [unwired: 2 out]
            }
            n164 = call "RefreshUI Event.vi"("Refresh (T)"=TRUE, "error in (no error)"=w313, "References in"=w309) -> ("error out"=w306:errorcluster)  [unwired: 7 in, 1 out]
            n165 = Unbundle By Name(w309) -> ("node change"=w308:T3)
            n166 = Generate User Event(user event=w308, event data cluster=w307, error in=w306) -> (error out=w305:errorcluster)  [unwired: 1 in, 1 out]
          }
          event "Timeout (us)": Value Change {
            n167 = event-data() -> ("NewVal"=w324:u32)  [unwired: 1 in]
            n168 = Unbundle By Name(w325) -> ("Node Ref"=w321:refnum<data-value>)
            n169 = in-place {
              in-place-border: w324 -> [w329]
              in-place-border: [w333] -> w327
              # "Store microsecond timeout value."
              n170 = in-place-dvr #11(w321) -> (w331:refnum<class "module editor node.lvclass">)  [unwired: 1 out]
              n171 = Divide(x=w329, y=1000000.0) -> (x/y=w328:dbl)
              n172 = call "write sync timeout.vi"("sync timeout"=w328, "shared memory editor node"=w331) -> ("error out"=w333:errorcluster, "shared memory editor node out"=w332:refnum<class "module editor node.lvclass">)  [unwired: 8 in]
              n173 = in-place-dvr #11(w332) -> ()  [unwired: 2 out]
            }
            n174 = call "RefreshUI Event.vi"("Refresh (T)"=TRUE, "error in (no error)"=w327, "References in"=w323) -> ("error out"=w320:errorcluster)  [unwired: 7 in, 1 out]
            n175 = Unbundle By Name(w323) -> ("node change"=w322:T3)
            n176 = Generate User Event(user event=w322, event data cluster=w321, error in=w320) -> (error out=w319:errorcluster)  [unwired: 1 in, 1 out]
          }
          event "output file path": Value Change {
            n177 = event-data() -> ("NewVal"=w339:path)  [unwired: 1 in]
            n178 = Unbundle By Name(w340) -> ("Node Ref"=w334:refnum<data-value>)
            n179 = in-place {
              in-place-border: w339 -> [w344]
              in-place-border: [w343] -> w341
              # "Replace the C header file directory destination in the module configuration."
              n180 = in-place-dvr #12(w334) -> (w346:refnum<class "module editor node.lvclass">)  [unwired: 1 out]
              n181 = call "write C header file path.vi"("c header file path"=w344, "shared memory editor node"=w346) -> ("error out"=w343:errorcluster, "shared memory editor node out"=w345:refnum<class "module editor node.lvclass">)  [unwired: 8 in]
              n182 = in-place-dvr #12(w345) -> ()  [unwired: 2 out]
            }
            n183 = call "RefreshUI Event.vi"("Refresh (T)"=TRUE, "error in (no error)"=w341, "References in"=w337) -> ("error out"=w336:errorcluster)  [unwired: 7 in, 1 out]
            n184 = Unbundle By Name(w337) -> ("node change"=w338:T3)
            n185 = Generate User Event(user event=w338, event data cluster=w334, error in=w336) -> (error out=w335:errorcluster)  [unwired: 1 in, 1 out]
          }
          event Value Change {
            n186 = event-data() -> ()  [unwired: 1 in, 1 out]
            n187 = Unbundle By Name(w362) -> ("engine"=w348:refnum<data-value>, "Node Ref"=w349:refnum<data-value>)
            n188 = Select(t=channel_classification."processing result" ("channel classification"), s="add from", f=channel_classification."processing parameter" ("channel classification")) -> (s? t:f=w352:T28)
            n189 = Unbundle By Name(w347) -> ("avail tags"=w354:refnum<vi>)
            n190 = call "get available list item.vi"("available tags list"=w354) -> ("error out"=w364:errorcluster, "data type"=w351:T2, "element name"=w353:string)  [unwired: 8 in]
            n191 = call "add list channel to configuration.vi"("channel classification"=w352, "element name"=w353, "error in (no error)"=w364, "data type"=w351, "node ref"=w349, "engine ref"=w348) -> ("error out"=w350:errorcluster)  [unwired: 5 in]
            n192 = Unbundle By Name(w360) -> ("node change"=w361:T3)
            n193 = call "RefreshUI Event.vi"("Refresh (T)"=TRUE, "error in (no error)"=w350, "References in"=w360) -> ("error out"=w359:errorcluster)  [unwired: 7 in, 1 out]
            n194 = Generate User Event(user event=w361, event data cluster=w349, error in=w359) -> (error out=w358:errorcluster)  [unwired: 1 in, 1 out]
          }
          event Value Change {
            n195 = event-data() -> ()  [unwired: 1 in, 1 out]
            n196 = Unbundle By Name(w380) -> ("engine"=w368:refnum<data-value>, "Node Ref"=w367:refnum<data-value>)
            n197 = Unbundle By Name(w375) -> ("from shm list"=w374:refnum<vi>, "to shm list"=w373:refnum<vi>)
            n198 = Select(t=w374, s="remove from", f=w373) -> (s? t:f=w371:refnum<vi>)
            n199 = call "get selected list item.vi"("ListBox in"=w371) -> ("error out"=w370:errorcluster, "valid selection?"=w366:bool, "element name"=w369:string)  [unwired: 8 in]
            n200 = case shown="True" w366 {
              tunnel: w370 -> [w382 w387]
              tunnel: w369 -> [_ w385]
              tunnel: w368 -> [_ w384]
              tunnel: w367 -> [_ w386]
              tunnel: [w382 w383] -> w365
              frame False {
              }
              frame True {
                n201 = call "remove list channel to configuration.vi"("error in (no error)"=w387, "element name"=w385, "node ref"=w386, "engine ref"=w384) -> ("error out"=w383:errorcluster)  [unwired: 7 in]
              }
            }
            n202 = Unbundle By Name(w378) -> ("node change"=w379:T3)
            n203 = call "RefreshUI Event.vi"("Refresh (T)"=TRUE, "error in (no error)"=w365, "References in"=w378) -> ("error out"=w377:errorcluster)  [unwired: 7 in, 1 out]
            n204 = Generate User Event(user event=w379, event data cluster=w367, error in=w377) -> (error out=w376:errorcluster)  [unwired: 1 in, 1 out]
          }
          event "major": Value Change {
            n205 = event-data() -> ("NewVal"=w394:u16)  [unwired: 1 in]
            n206 = Unbundle By Name(w395) -> ("Node Ref"=w389:refnum<data-value>)
            n207 = in-place {
              in-place-border: w394 -> [w397]
              in-place-border: [w399] -> w388
              # "Update major revision number."
              n208 = in-place-dvr #13(w389) -> (w401:refnum<class "module editor node.lvclass">, w400:errorcluster)
              n209 = call "write revision major.vi"("error in"=w400, "revision major"=w397, "shared memory editor node"=w401) -> ("error out"=w399:errorcluster, "shared memory editor node out"=w398:refnum<class "module editor node.lvclass">)  [unwired: 7 in]
              n210 = in-place-dvr #13(w398) -> ()  [unwired: 2 out]
            }
            n211 = call "RefreshUI Event.vi"("Refresh (T)"=TRUE, "error in (no error)"=w388, "References in"=w392) -> ("error out"=w390:errorcluster)  [unwired: 7 in, 1 out]
            n212 = Unbundle By Name(w392) -> ("node change"=w393:T3)
            n213 = Generate User Event(user event=w393, event data cluster=w389, error in=w390) -> (error out=w391:errorcluster)  [unwired: 1 in, 1 out]
          }
          event "minor": Value Change {
            n214 = event-data() -> ("NewVal"=w408:u16)  [unwired: 1 in]
            n215 = Unbundle By Name(w409) -> ("Node Ref"=w403:refnum<data-value>)
            n216 = in-place {
              in-place-border: w408 -> [w411]
              in-place-border: [w415] -> w402
              # "Update major revision number."
              n217 = in-place-dvr #14(w403) -> (w413:refnum<class "module editor node.lvclass">, w412:errorcluster)
              n218 = call "write revision minor.vi"("error in"=w412, "revision minor"=w411, "shared memory editor node"=w413) -> ("error out"=w415:errorcluster, "shared memory editor node out"=w414:refnum<class "module editor node.lvclass">)  [unwired: 7 in]
              n219 = in-place-dvr #14(w414) -> ()  [unwired: 2 out]
            }
            n220 = call "RefreshUI Event.vi"("Refresh (T)"=TRUE, "error in (no error)"=w402, "References in"=w406) -> ("error out"=w404:errorcluster)  [unwired: 7 in, 1 out]
            n221 = Unbundle By Name(w406) -> ("node change"=w407:T3)
            n222 = Generate User Event(user event=w407, event data cluster=w403, error in=w404) -> (error out=w405:errorcluster)  [unwired: 1 in, 1 out]
          }
          event "Generate Header": Value Change {
            # "/<C header file directory/<ConfigurationFileName>_<FileString>.h"
            n223 = event-data() -> ()  [unwired: 1 in, 1 out]
            n224 = Unbundle By Name(w425) -> ("engine"=w417:refnum<data-value>, "Node Ref"=w424:refnum<data-value>)
            n225 = in-place {
              in-place-border: [w436] -> w422
              # "Generate the C header file."
              n226 = in-place-dvr #15(w417) -> (w431:refnum<class "Engine Parent Editor Node.lvclass">, w428:errorcluster)
              n227 = in-place-dvr #16(w424) -> (w426:refnum<class "module editor node.lvclass">, w429:errorcluster)
              n228 = Merge Errors(w428, w429) -> (w427:errorcluster)
              n229 = call "read c header file path.vi"("error in"=w427, "shared memory editor node"=w426) -> ("error out"=w435:errorcluster, "c header file path"=w433:path, "shared memory editor node out"=w434:refnum<class "module editor node.lvclass">)  [unwired: 7 in]
              n230 = Empty String/Path?(string/path=w433) -> (empty?=w432:bool)
              n231 = case shown="False" w432 {
                tunnel: [w445 w450] -> w437
                tunnel: [w438 w451] -> w436
                tunnel: w435 -> [w444 w451]
                tunnel: w434 -> [w443 w450]
                tunnel: w433 -> [w442 _]
                tunnel: [w440 w448] -> w430
                tunnel: w431 -> [w441 w448]
                frame False {
                  n232 = call "generate header file.vi"("engine in"=w441, "error in (no error)"=w444, "file path"=w442, "shared memory editor node in"=w443) -> ("error out"=w439:errorcluster, "shared memory editor node out"=w445:refnum<class "module editor node.lvclass">, "engine out"=w440:refnum<class "Engine Parent Editor Node.lvclass">)  [unwired: 4 in, 1 out]
                  n233 = case shown="No Error" w439 {
                    selector: w439 -> [_ w447]
                    tunnel: [_ w447] -> w438
                    frame No Error {
                      n234 = One Button Dialog(message="Success!") -> ()  [unwired: 1 in, 1 out]
                    }
                    frame Error {
                    }
                  }
                }
                frame True {
                  n235 = One Button Dialog(message="Please enter a valid file path.") -> ()  [unwired: 1 in, 1 out]
                }
              }
              n236 = in-place-dvr #15(w430) -> (w416:errorcluster)  [unwired: 1 out]
              n237 = in-place-dvr #16(w437) -> (w423:errorcluster)  [unwired: 1 out]
            }
            n238 = Merge Errors(w416, w423, w422) -> (w419:errorcluster)
            n239 = call "RefreshUI Event.vi"("Refresh (T)"=TRUE, "error in (no error)"=w419, "References in"=w420) -> ("error out"=w418:errorcluster)  [unwired: 7 in, 1 out]
          }
          event Panel Close? {
            n240 = event-data() -> ()  [unwired: 1 in, 1 out]
            n241 = Unbundle By Name(w453) -> ("stop event"=w452:T6)
            n242 = Generate User Event(user event=w452, event data cluster=TRUE ("event data")) -> ()  [unwired: 2 in, 2 out]
            n243 = event-data("Discard?"=TRUE) -> ()  [unwired: 1 in, 1 out]
          }
          event Value Change {
            n244 = event-data() -> ()  [unwired: 1 in, 1 out]
            n245 = call "Add New Line.vi"("objects"=w462) -> ("error out"=w460:errorcluster, "success"=w458:bool)  [unwired: 8 in, 1 out]
            n246 = call "Node Change Event.vi"("error in (no error)"=w460, "Send (T)"=w458, "objects"=w462, "References in"=w461) -> ("error out"=w459:errorcluster)  [unwired: 7 in]
            n247 = call "RefreshUI Event.vi"("error in (no error)"=w459, "References in"=w461) -> ("error out"=w457:errorcluster)  [unwired: 8 in, 1 out]
          }
          event Value Change {
            n248 = event-data() -> ()  [unwired: 1 in, 1 out]
            n249 = call-dynamic "Active Line Name.vi"("Multi Column Listbox in"=w470) -> ("error out"=w468:errorcluster, "Active Line Name"=w469:string)  [unwired: 8 in, 1 out]
            n250 = call "Remove Line.vi"("error in"=w468, "Active Line Name"=w469, "Objects"=w474) -> ("error out"=w471:errorcluster)  [unwired: 8 in]
            n251 = call "RefreshUI Event.vi"("error in (no error)"=w471, "References in"=w475) -> ("error out"=w473:errorcluster, "References out"=w472:T21)  [unwired: 8 in]
            n252 = call "Node Change Event.vi"("error in (no error)"=w473, "objects"=w474, "References in"=w472) -> ("error out"=w465:errorcluster)  [unwired: 8 in]
            n253 = property on="Table" class="MCListbox (strict)"(error in=w465) -> (error out=w463:errorcluster, "Value"=w466:i32)  [unwired: 1 in, 1 out]
            n254 = Decrement(x=w466) -> (x-1=w467:i32)
            n255 = property on="Table" class="MCListbox (strict)"(error in=w463, "Val(Sgnl)"=w467) -> (error out=w464:errorcluster)  [unwired: 1 in, 1 out]
          }
          event Value Change {
            n256 = event-data() -> ()  [unwired: 1 in, 1 out]
            n257 = call-dynamic "Active Line Name.vi"("Multi Column Listbox in"=w480) -> ("error out"=w477:errorcluster, "Active Line Name"=w478:string)  [unwired: 8 in, 1 out]
            n258 = call "Edit Line.vi"("error in"=w477, "Line Name"=w478, "References"=w479) -> ("error out"=w482:errorcluster, "change?"=w476:bool)  [unwired: 7 in]
            n259 = call "Node Change Event.vi"("error in (no error)"=w482, "Send (T)"=w476, "objects"=w479, "References in"=w483) -> ("error out"=w481:errorcluster)  [unwired: 7 in]
          }
          event User Event {
            n260 = event-data() -> ("Selected Value"=w491:string, "Line Name"=w488:string)  [unwired: 1 in]
            n261 = case shown="\"Add\"" w491 {
              tunnel: w488 -> [w494 _ w500]
              tunnel: w486 -> [w493 w496 w499]
              tunnel: [w492 w495 w498] -> w487
              tunnel: [_ _ w497] -> w484
              frame "Remove" {
                n262 = call "Remove Line.vi"("Active Line Name"=w494, "Objects"=w493) -> ("error out"=w492:errorcluster)  [unwired: 9 in]
              }
              frame "Add" {
                n263 = call "Add New Line.vi"("objects"=w496) -> ("error out"=w495:errorcluster)  [unwired: 8 in, 2 out]
              }
              frame "Edit", Default {
                n264 = call "Edit Line.vi"("Line Name"=w500, "References"=w499) -> ("error out"=w498:errorcluster, "change?"=w497:bool)  [unwired: 8 in]
              }
            }
            n265 = call "Node Change Event.vi"("error in (no error)"=w487, "Send (T)"=w484, "objects"=w486, "References in"=w485) -> ("error out"=w490:errorcluster)  [unwired: 7 in]
            n266 = call "RefreshUI Event.vi"("error in (no error)"=w490, "References in"=w485) -> ("error out"=w489:errorcluster)  [unwired: 8 in, 1 out]
          }
          event "Table": Value Change {
            # "Disable these when nothing in the table is selected."
            n267 = event-data() -> ("NewVal"=w506:i32)  [unwired: 1 in]
            n268 = Equal?(x=w506, y=-1) -> (x = y?=w504:bool)
            n269 = Select(t=T29."Disabled and Grayed Out" ("Disabled"), s=w504, f=T29."Enabled") -> (s? t:f=w502:T29)
            n270 = property on="Remove Button" class="Bool"("DisabledEnum"=w502) -> ()  [unwired: 2 in, 2 out]
            n271 = property on="settings" class="Bool"("DisabledEnum"=w502) -> ()  [unwired: 2 in, 2 out]
          }
        }
        n272 = call "Local Error Handler.vi"("error in"=w81, "Stop in"=w83) -> ("error out"=w82:errorcluster, "Stop out"=w84:bool)  [unwired: 8 in]
      }
      n273 = disable-structure shown="Disabled" {
        disable-tunnel: w68 -> [w74 _]
        disable-tunnel: [w73 _] -> w67
        frame Disabled {
          n274 = call-dynamic "Event Handler.vi"("Listbox in"=w74) -> ("error out"=w73:errorcluster)  [unwired: 9 in, 1 out]
        }
        frame Enabled {
        }
      }
      n275 = Merge Errors(w66, w67) -> (w65:errorcluster)
    }
    frame Error {
    }
  }
  n276 = Unregister For Events(event registration refnum=w60, error in=w59) -> (error out=w58:errorcluster)
  n277 = call <vilib>:"Simple Error Handler.vi"("error in (no error)"=w58) -> ()  [unwired: 4 in, 5 out]
